vi "Dep.vi"(0 "x":dbl) -> (4 "y":dbl)   [LabVIEW 2026]
doc: "Test fixture: adds one."
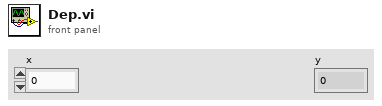
[diagram p1: front panel]
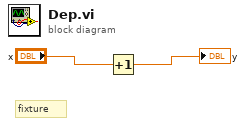
[diagram p0: block diagram]
diagram:
  # "fixture"
  n1 = Increment(x="x") -> (x+1=→"y":dbl)
